vi "Create New Handler.File.Text.vi"(6 "File Path":path, 7 "Handler.File.Text in":refnum<class "Handler.File.Text.lvclass">, 8 "error in (no error)":errorcluster, 10 "Name":string, 11 "Level":T1(ring)) -> (0 "error out":errorcluster, 3 "Handler.File.Text out":refnum<class "Handler.File.Text.lvclass">)   [LabVIEW 2017, in "Error Log.lvlib" / "Handler.File.Text.lvclass"]
uses:
  Handler.File.Text.lvclass
  \\192.168.1.40\Neosoft/Partage/Dossiers Personnels/BRO/DevTools_BR/wc/ErrorLog/src/Handler.File/Handler.File.lvclass
  <vilib>/Utility/error.llb/Error Cluster From Error Code.vi
  <vilib>/ErrorRing/Error Ring.xnode
  Handler.File/Handler.File.lvclass
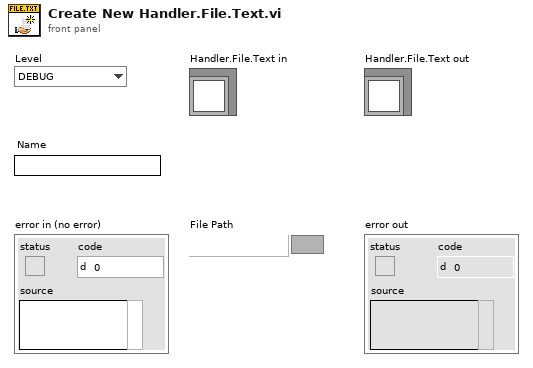
[diagram p1: front panel]
types:
  T1 = enum16{"DEBUG", "INFO", "WARNING", "ERROR", "CRITICAL"}
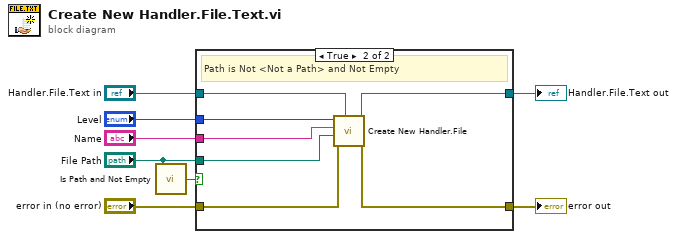
[diagram p0: block diagram]
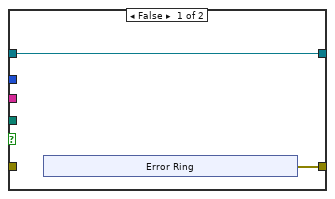
[diagram p2: hidden frame]
diagram:
  n1 = call <vilib>:"Is Path and Not Empty.vi"("path"="File Path") -> ("Is Path and Not Empty?"=w2:bool)  [unwired: 4 in]
  n2 = case shown="True" w2 {
    tunnel: "Handler.File.Text in" -> [w10 w21]
    tunnel: [w10 w20] -> w7
    tunnel: "error in (no error)" -> [_ w19]
    tunnel: [w9 w18] -> w5
    tunnel: "File Path" -> [_ w17]
    tunnel: "Name" -> [_ w16]
    tunnel: "Level" -> [_ w15]
    frame False {
      n3 = xnode "Error Ring"() -> ("error out"=w9:errorcluster)
    }
    frame True {
      # "Path is Not <Not a Path> and Not Empty"
      n4 = call "Create New Handler.File.vi"("Handler.File in"=w21, "error in (no error)"=w19, "File Path"=w17, "Name"=w16, "Level"=w15) -> ("error out"=w18:errorcluster, "Handler.File out"=w20:refnum<class "Handler.File.Text.lvclass">)  [unwired: 5 in]
    }
  }
  "error out" <- w5
  "Handler.File.Text out" <- w7
